vi "FX_WriteD.vi"(8 "error in (no error)":errorcluster, 9 "Value":u16, 10 "D":u16, 11 "VISA in":refnum<visa-resource-name>) -> (2 "error out":errorcluster, 3 "VISA out":refnum<visa-resource-name>)   [LabVIEW 2018]
doc: "Use this template to build a VI to use as a subVI."
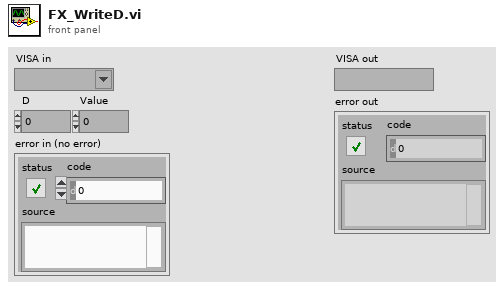
[diagram p1: front panel]
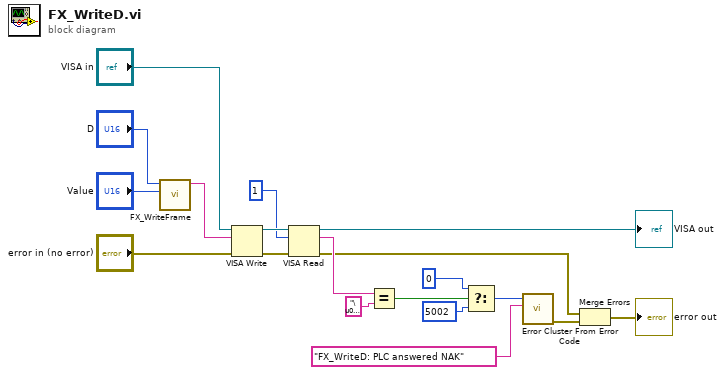
[diagram p0: block diagram]
diagram:
  n1 = call "FX_WriteFrame.vi"("Value"="Value", "D"="D") -> ("Frame"=w16:string)  [unwired: 9 in]
  n2 = VISA Write(VISA resource name="VISA in", write buffer=w16, error in (no error)="error in (no error)") -> (VISA resource name out=w14:refnum<visa-resource-name>, error out=w13:errorcluster)  [unwired: 1 out]
  n3 = VISA Read(VISA resource name=w14, byte count=u32 1, error in (no error)=w13) -> (VISA resource name out=→"VISA out":refnum<visa-resource-name>, read buffer=w11:string, error out=w4:errorcluster)  [unwired: 1 out]
  n4 = Equal?(x=w11, y="\u0006") -> (x = y?=w9:bool)
  n5 = Select(t=0, s=w9, f=5002) -> (s? t:f=w6:i32)
  n6 = call <vilib>:"Error Cluster From Error Code.vi"("error message (\"\")"="FX_WriteD: PLC answered NAK", "error code (0)"=w6) -> ("error out"=w3:errorcluster)  [unwired: 7 in]
  n7 = Merge Errors(w4, w3) -> (→"error out":errorcluster)
